vi "front.vi"() -> ()   [LabVIEW 2015]
panel:
  in  "stop":bool
  out "destIndicator":u8
  out "downIndicator":bool
  out "upIndicator":bool
  out "etageIndicator":u8
  out "porteIndicator":string
  out "Alarme":bool
  in  "Etage 2":bool
  in  "RDC":bool
  in  "Etage 1":bool
  # "Destination"
  # "Actuel"
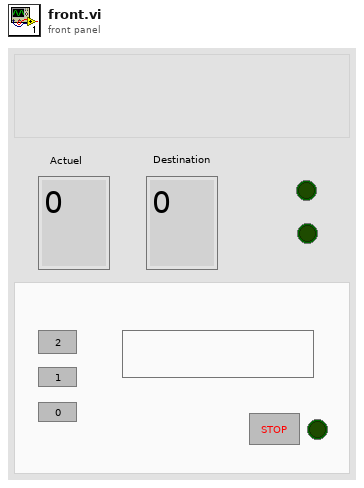
[diagram p1: front panel]
types:
  T1 = enum16{"INIT", "ATTENTE", "DEPLACEMENT", "PORTE_OUVERTE", "PORTE_FERMEE", "ARRET_URGENCE"}
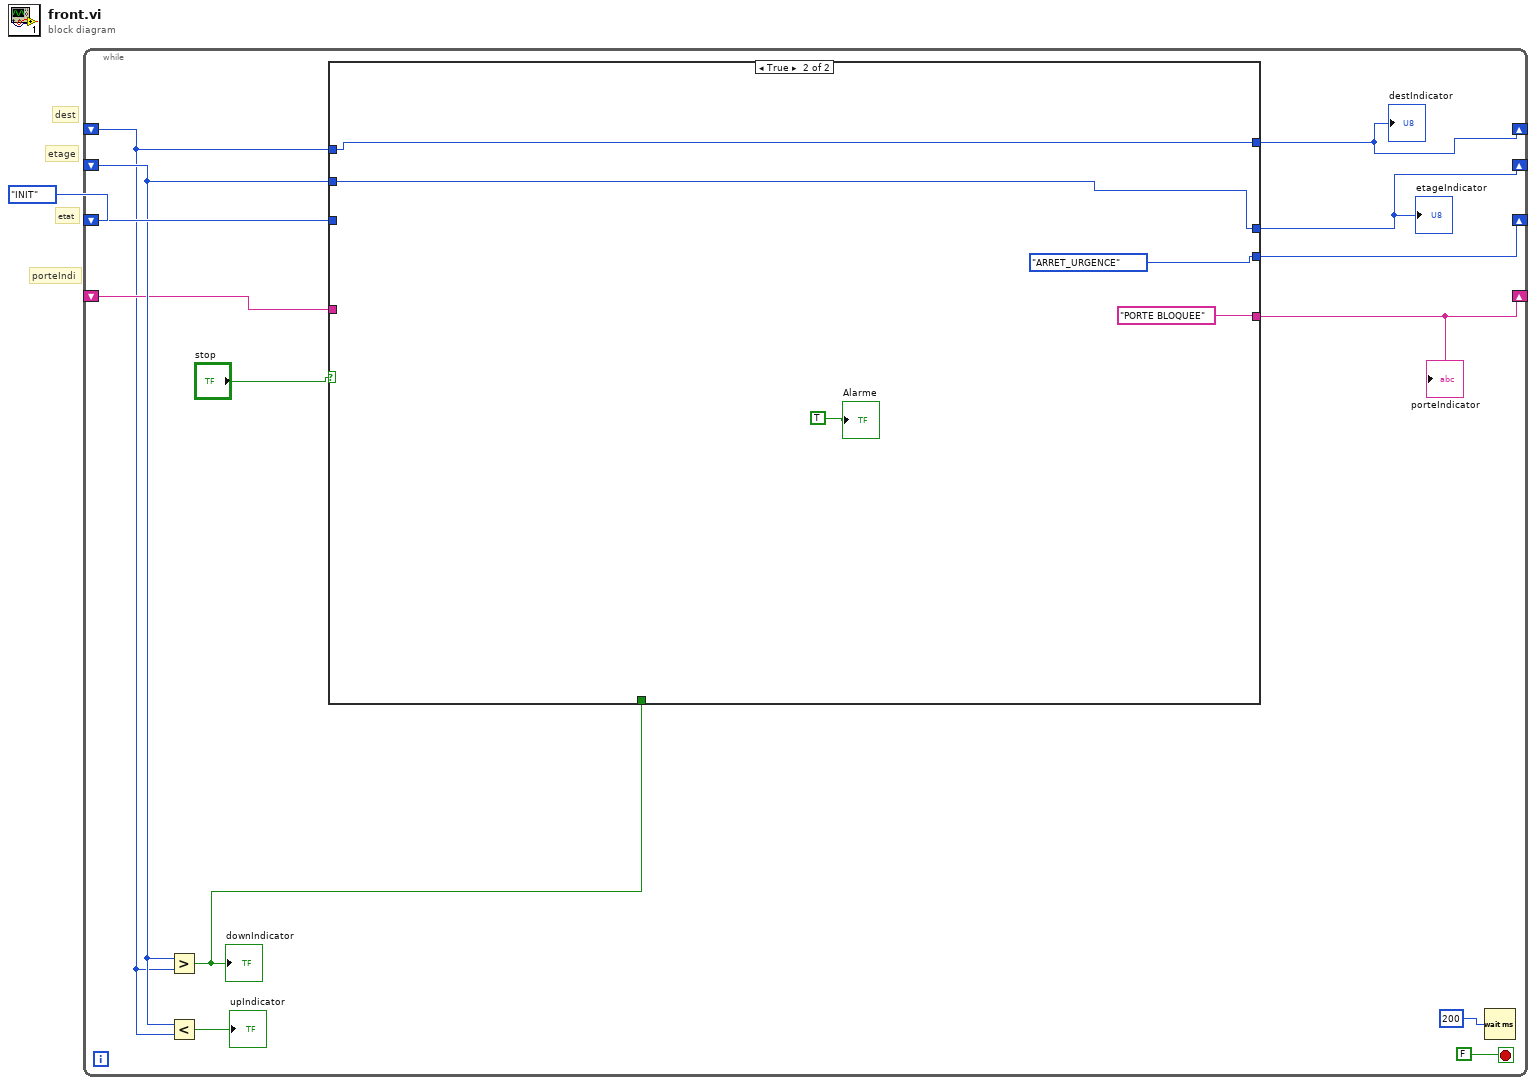
[diagram p0: block diagram]
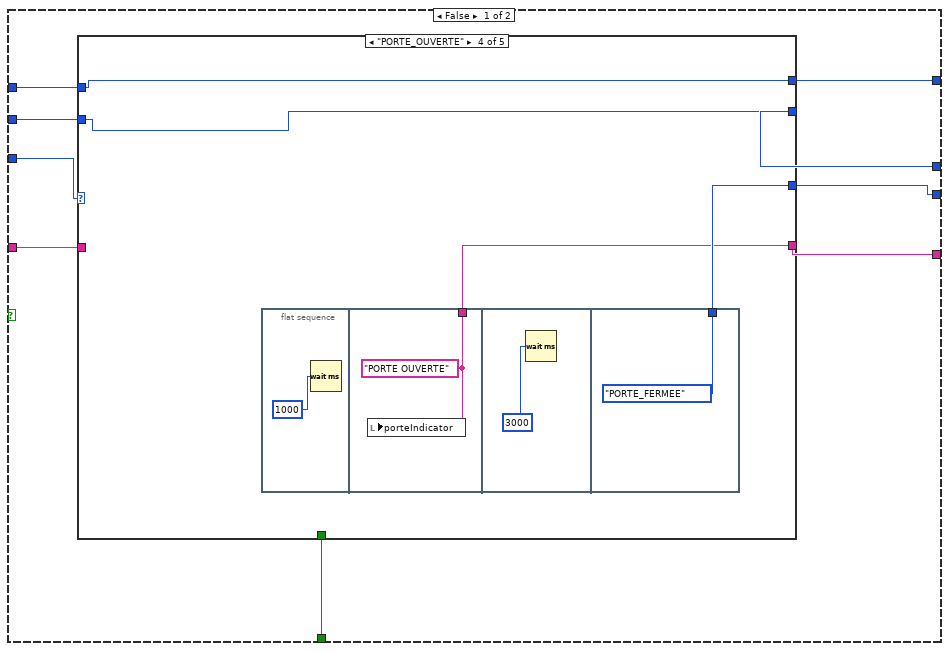
[diagram p2: hidden frame]
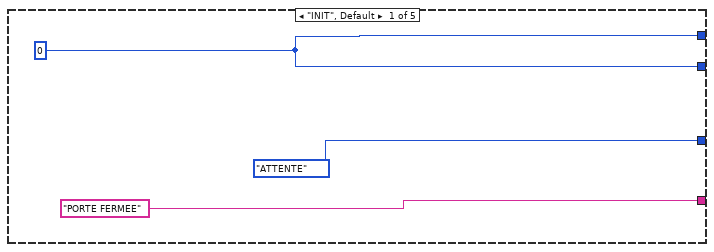
[diagram p3: hidden frame]
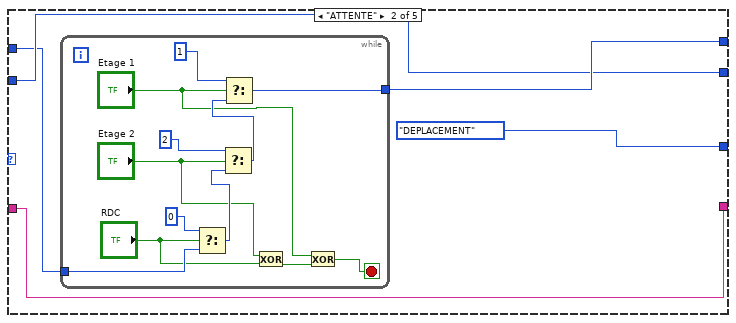
[diagram p4: hidden frame]
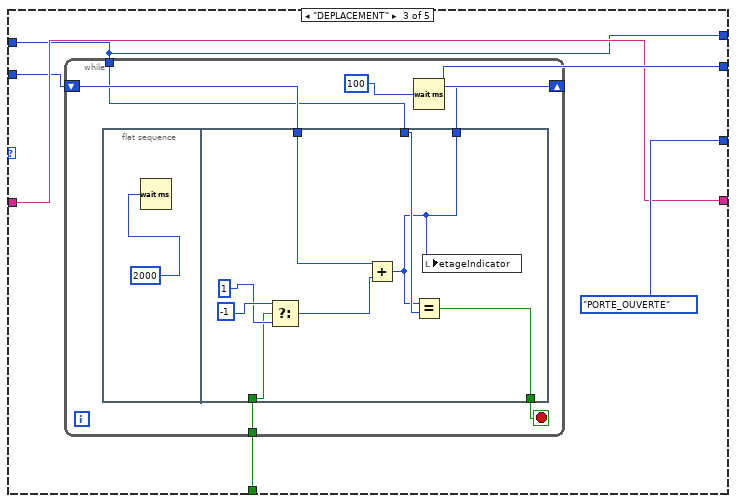
[diagram p5: hidden frame]
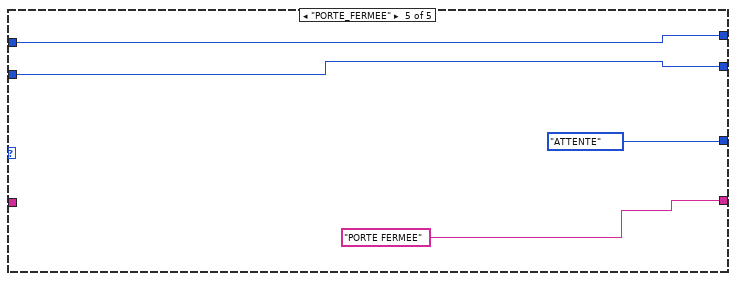
[diagram p6: hidden frame]
diagram:
  # "porteIndi"
  # "etat"
  # "dest"
  # "etage"
  n1 = while {
    shift-right: [w12] -> _
    shift-left: T1."INIT" ("Etats") -> [w13]
    shift-right: [w9] -> _
    shift-left: _ -> [w4]
    shift-right: [w8] -> _
    shift-left: _ -> [w7]
    shift-right: [w6] -> _
    shift-left: _ -> [w5]
    stop <- FALSE stop-if-true
    n2 = Greater?(x=w7, y=w4) -> (0:w11:bool)
    "downIndicator" <- w11
    n3 = Less?(x=w7, y=w4) -> (x < y?=→"upIndicator":bool)
    n4 = case shown="True" "stop" {
      tunnel: w13 -> [w23 _]
      tunnel: [w15 T1."ARRET_URGENCE" ("Etats")] -> w12
      tunnel: w11 -> [w22 _]
      tunnel: [w21 w80] -> w9
      tunnel: [w20 w79] -> w8
      tunnel: w7 -> [w19 w79]
      tunnel: [w18 "PORTE BLOQUEE"] -> w6
      tunnel: w5 -> [w17 _]
      tunnel: w4 -> [w16 w80]
      frame False {
        n5 = case shown="\"PORTE_OUVERTE\"" w23 {
          tunnel: [T1."ATTENTE" ("Etats") T1."DEPLACEMENT" ("Etats") T1."PORTE_OUVERTE" ("Etats") w66 T1."ATTENTE" ("Etats")] -> w15
          tunnel: [w24 w30 w48 w67 w75] -> w20
          tunnel: [w24 w31 w45 w68 w76] -> w21
          tunnel: w22 -> [_ _ w49 _ _]
          tunnel: ["PORTE FERMEE" w29 w46 w65 "PORTE FERMEE"] -> w18
          tunnel: w19 -> [_ w30 w44 w67 w75]
          tunnel: w17 -> [_ w29 w46 _ _]
          tunnel: w16 -> [_ w28 w45 w68 w76]
          frame "INIT", Default {
            w24 = u8 0
          }
          frame "ATTENTE" {
            n6 = while {
              tunnel: [w43] -> w31
              tunnel: w28 -> [w42]
              stop <- w32 stop-if-true
              n7 = Select(t=u8 0, s="RDC", f=w42) -> (s? t:f=w38:u8)
              n8 = Select(t=u8 2, s="Etage 2", f=w38) -> (s? t:f=w37:u8)
              n9 = Select(t=u8 1, s="Etage 1", f=w37) -> (s? t:f=w43:u8)
              n10 = Exclusive Or(1:"RDC", 2:"Etage 2") -> (0:w34:bool)
              n11 = Exclusive Or(1:w34, 2:"Etage 1") -> (0:w32:bool)
            }
          }
          frame "DEPLACEMENT" {
            n12 = while {
              tunnel: w49 -> [w55]
              tunnel: w45 -> [w52]
              shift-right: [w51] -> w48
              shift-left: w44 -> [w53]
              stop <- w54 stop-if-true
              n13 = flat-sequence {
                tunnel: w55 -> [w61]
                tunnel: [w60] -> w54
                tunnel: w53 -> [w59]
                tunnel: w52 -> [w58]
                tunnel: [w57] -> w51
                frame #0 {
                  n14 = Wait (ms)(milliseconds to wait=u32 2000) -> ()  [unwired: 1 out]
                }
                frame #1 {
                  n15 = Select(t=i8 -1, s=w61, f=u8 1) -> (s? t:f=w62:u8)
                  n16 = Add(x=w59, y=w62) -> (x+y=w57:u8)
                  n17 = Equal?(x=w57, y=w58) -> (x = y?=w60:bool)
                  n18 = local write "etageIndicator"(w57) -> ()
                }
              }
              n19 = Wait (ms)(milliseconds to wait=u32 100) -> ()  [unwired: 1 out]
            }
          }
          frame "PORTE_OUVERTE" {
            n20 = flat-sequence {
              tunnel: [w70] -> w65
              tunnel: [T1."PORTE_FERMEE" ("Etats")] -> w66
              frame #0 {
                n21 = Wait (ms)(milliseconds to wait=u32 1000) -> ()  [unwired: 1 out]
              }
              frame #1 {
                w70 = "PORTE OUVERTE"
                n22 = local write "porteIndicator"(w70) -> ()
              }
              frame #2 {
                n23 = Wait (ms)(milliseconds to wait=u32 3000) -> ()  [unwired: 1 out]
              }
              frame #3 {
              }
            }
          }
          frame "PORTE_FERMEE" {
          }
        }
      }
      frame True {
        "Alarme" <- TRUE
      }
    }
    "porteIndicator" <- w6
    "etageIndicator" <- w8
    "destIndicator" <- w9
    n24 = Wait (ms)(milliseconds to wait=u32 200) -> ()  [unwired: 1 out]
  }
